vi "Frame Order 3.vi"() -> ()   [LabVIEW 2026]
doc: "Probe three: a stacked sequence with a case in its middle frame."
panel:
  in  "c":string="u"
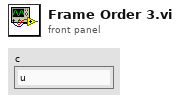
[diagram p1: front panel]
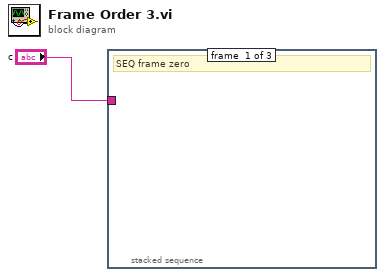
[diagram p0: block diagram]
diagram:
  n1 = stacked-sequence {
    tunnel: "c" -> [_ w2 _]
    frame #0 {
      # "SEQ frame zero"
    }
    frame #1 {
      # "SEQ frame one"
      n2 = case shown="\"b\", Default" w2 {
        frame "u" {
          # "CASE frame u"
        }
        frame Default {
          # "CASE frame default"
        }
      }
    }
    frame #2 {
      # "SEQ frame two"
    }
  }
